vi "Format Call Chain.vi"(5 "number of callers (-1: all)":i32=-1, 7 "delimiter (\" > \")":string=" > ", 9 "string length (-1: none)":i32=-1, 10 "remove namespaces? (T)":bool=TRUE, 11 "call chain":string[](array[string])) -> (3 "formatted call chain":string)   [LabVIEW 2018, in "GLog.lvlib" / "Format String.lvclass"]
uses:
  Format String.lvclass
  <vilib>/regexp/Match Regular Expression.xnode
  dependencies/Utilities/Utilities.lvlib
panel:
  # "Connector Pane"
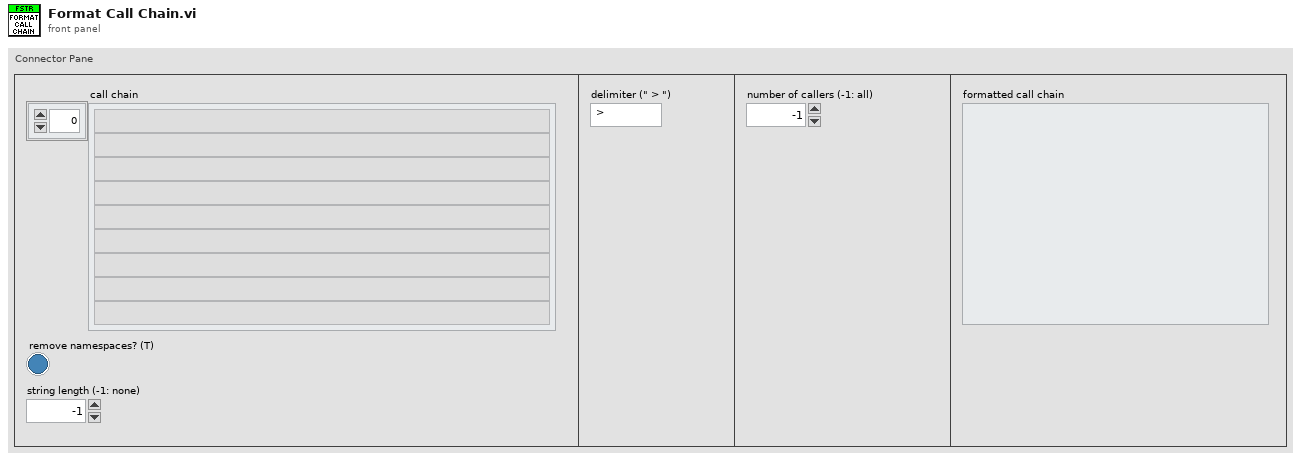
[diagram p1: front panel]
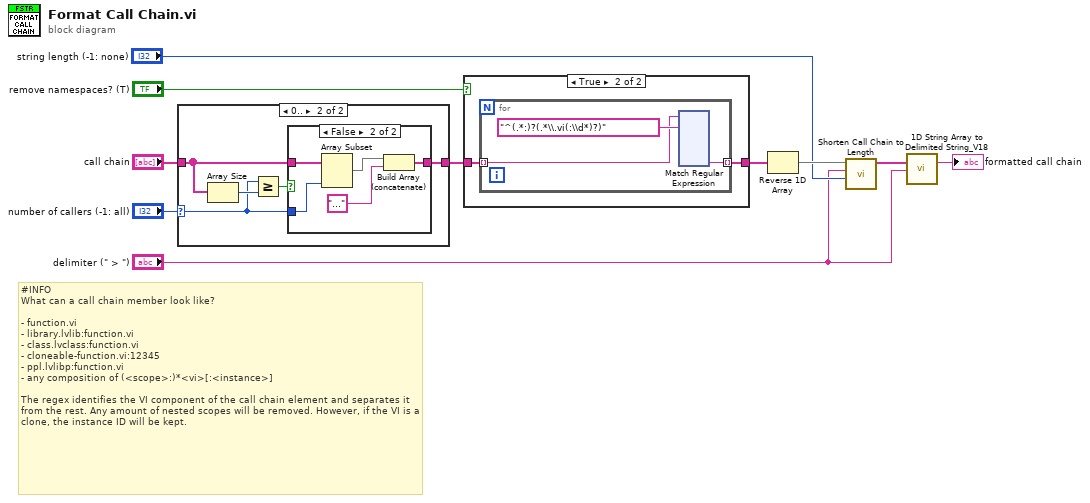
[diagram p0: block diagram]
diagram:
  # "#INFO\nWhat can a call chain member look like?\n\n- function.vi\n- library.lvlib:function.vi\n- class.lvclass:function.vi\n- cloneable-function.vi:12345\n- ppl.lvlibp:function.vi\n- any composition of (<scope>:)*<vi>[:<instance>]\n\nThe regex identifies the VI component of the call chain element and separates it from the rest. Any amount of nested scopes will be removed. However, if the VI is a clone, the instance ID will be kept."
  n1 = case shown="0.." "number of callers (-1: all)" {
    selector: "number of callers (-1: all)" -> [_ w13]
    tunnel: "call chain" -> [w11 w15]
    tunnel: [w11 w16] -> w3
    frame ..-1 {
    }
    frame 0.. {
      n2 = Array Size(array=w15) -> (size(s)=w14:i32)
      n3 = Greater Or Equal?(x=w13, y=w14) -> (x >= y?=w12:bool)
      n4 = case shown="False" w12 {
        tunnel: [w17 w19] -> w16
        tunnel: w15 -> [w17 w21]
        tunnel: w13 -> [_ w20]
        frame True {
        }
        frame False {
          n5 = Array Subset(array=w21, length=w20) -> (w22:string[])  [unwired: 1 in]
          n6 = Build Array (concatenate)(w22, "…" ("String")) -> (w19:string[])
        }
      }
    }
  }
  n7 = case shown="True" "remove namespaces? (T)" {
    tunnel: w3 -> [w23 w25]
    tunnel: [w23 w24] -> w10
    frame False {
    }
    frame True {
      n8 = for {
        tunnel: w25 -> [w27] mode=indexing
        tunnel: [w26] -> w24 mode=indexing
        n9 = xnode "Match Regular Expression"("input string"=w27, "regular expression"="^(.*:)?(.*\\.vi(:\\d*)?)") -> ("submatch 2"=w26:string)  [unwired: 4 in, 6 out]
      }
    }
  }
  n10 = Reverse 1D Array(array=w10) -> (reversed array=w6:string[])
  n11 = call "Shorten Call Chain to Length.vi"("desired length"="string length (-1: none)", "delimiter"="delimiter (\" > \")", "call chain in"=w6) -> ("call chain out"=w7:string[])  [unwired: 8 in]
  n12 = call "1D String Array to Delimited String_V18.vi"("delimiter"="delimiter (\" > \")", "string array"=w7) -> ("delimited string"=→"formatted call chain":string)  [unwired: 9 in]
